vi "decoder.vi"() -> ()   [LabVIEW 2025]
panel:
  out "Message":u32 format="%b"
  in  "Stop":bool
  in  "P":u32 format="%b"
  out "maska":u32 format="%b"
  out "Checksum":u32 format="%b"
  in  "Message with CRC":u32 format="%b"
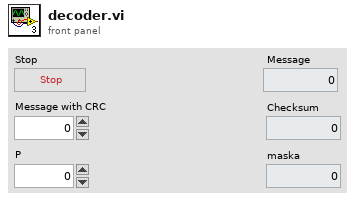
[diagram p1: front panel]
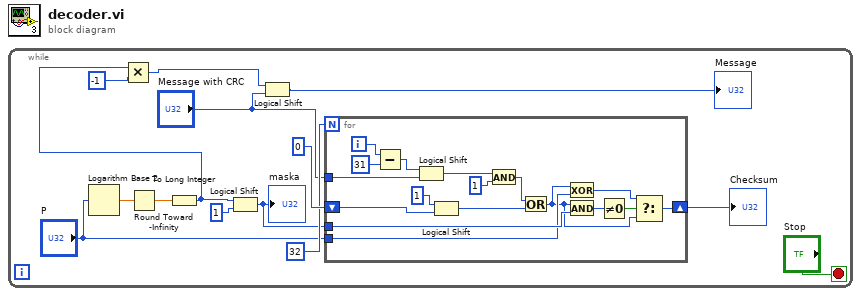
[diagram p0: block diagram]
diagram:
  n1 = while {
    stop <- "Stop" stop-if-true
    n2 = Logarithm Base 2(1:"P") -> (0:w13:dbl)
    n3 = Round Toward -Infinity(1:w13) -> (0:w12:dbl)
    n4 = To Long Integer(number=w12) -> (32bit integer=w5:i32)
    n5 = Multiply(x=w5, y=-1) -> (x*y=w3:i32)
    n6 = Logical Shift(y=w5, x=u32 1) -> (x << y=w7:u32)
    "maska" <- w7
    n7 = Logical Shift(y=w3, x="Message with CRC") -> (x << y=→"Message":u32)
    n8 = for {
      N: 32 -> [_]
      shift-right: [w15] -> w6
      shift-left: u32 0 -> [w25]
      tunnel: "Message with CRC" -> [w31]
      tunnel: "P" -> [w18]
      tunnel: w7 -> [w21]
      i -> [w30]
      n9 = Subtract(x=w30, y=31) -> (x-y=w28:i32)
      n10 = Logical Shift(y=w28, x=w31) -> (x << y=w27:u32)
      n11 = Logical Shift(y=i16 1, x=w25) -> (x << y=w23:u32)
      n12 = And(x=w27, y=u32 1) -> (x .and. y?=w22:u32)
      n13 = Or(x=w22, y=w23) -> (x .or. y?=w16:u32)
      n14 = Exclusive Or(1:w18, 2:w16) -> (0:w17:u32)
      n15 = And(x=w16, y=w21) -> (x .and. y?=w20:u32)
      n16 = Not Equal To 0?(x=w20) -> (x != 0?=w19:bool)
      n17 = Select(t=w17, s=w19, f=w16) -> (s? t:f=w15:u32)
    }
    "Checksum" <- w6
  }
